vi "Stop Pat GV.vi"() -> ()   [LabVIEW 2020]
panel:
  in  "Stop Pat":bool
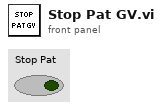
[diagram p1: front panel]
diagram:
